vi "make channel name_extract_priv_method.vi"(8 "error in (no error)":errorcluster, 10 "channel name":string, 11 "group name":string) -> (0 "error out":errorcluster, 3 "qualified channel":string)   [LabVIEW 2020, in "Nominal-TDMS-Upload.lvlib" / "Nominal-TDMS-Upload.lvclass"]
uses:
  Nominal-TDMS-Upload.lvclass
  <vilib>/Nominal/Nominal IO Client/lv_src/Nominal Client/Nominal Client.lvclass
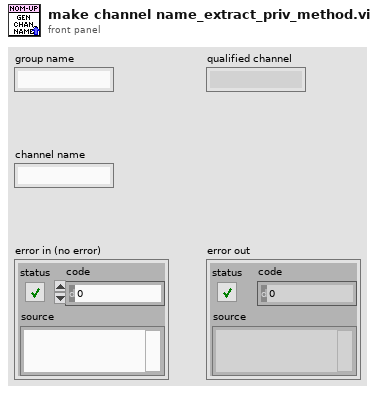
[diagram p1: front panel]
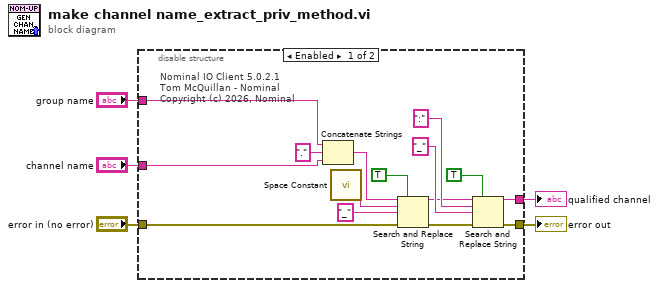
[diagram p0: block diagram]
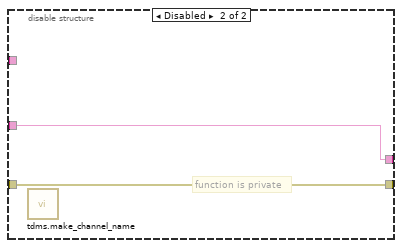
[diagram p2: hidden frame]
diagram:
  n1 = disable-structure shown="Enabled" {
    disable-tunnel: "group name" -> [w10 _]
    disable-tunnel: "channel name" -> [w9 w22]
    disable-tunnel: [w7 w22] -> w3
    disable-tunnel: "error in (no error)" -> [w8 w21]
    disable-tunnel: [w6 w21] -> w5
    frame Enabled {
      # "Nominal IO Client 5.0.2.1\nTom McQuillan - Nominal\nCopyright (c) 2026, Nominal"
      n2 = Concatenate Strings(w10, "." ("string"), w9) -> (w16:string)
      n3 = call <vilib>:"Space Constant.vi"() -> ("String"=w19:string)
      n4 = Search and Replace String(replace all?=TRUE ("replace all? (F)"), input string=w16, search string=w19, replace string="_", error in=w8) -> (result string=w12:string, error out=w11:errorcluster)  [unwired: 3 in, 2 out]
      n5 = Search and Replace String(replace all?=TRUE ("replace all? (F)"), input string=w12, search string=":", replace string="_", error in=w11) -> (result string=w7:string, error out=w6:errorcluster)  [unwired: 3 in, 2 out]
    }
    frame Disabled {
      # "function is private"
      n6 = call <vilib>:"tdms.make_channel_name.vi"() -> ()  [unwired: 10 in, 2 out]
    }
  }
  "error out" <- w5
  "qualified channel" <- w3
